vi "Make Counter Signal.vi"(11 "Node Ptr":T1=18446744073709551615 format="%.0x") -> ()   [LabVIEW 2025, in "Protection and Counter Addon System Explorer.lvlib"]
uses:
  Protection and Counter Addon System Explorer.lvlib
  Addon Shared/SubVIs/GUID Lookup.vi
  Addon Shared/Protection and Counter Addon Shared.lvlib
  SubModules/Frame-Protection-Support/Source/System Explorer/Protection and Counter Support System Explorer.lvlib
  SubModules/Frame-Protection-Support/Source/System Explorer/Types/Switch GUID Settings.ctl
  <vilib>/NI VeriStand/Custom Device API/Custom Device Item Ref.ctl
  <vilib>/NI VeriStand/Custom Device API/Custom Device API.lvlib
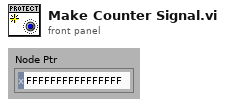
[diagram p1: front panel]
types:
  T1 = typedef "Custom Device API.lvlib/Custom Device Item Ref.ctl" = u64
  T2 = typedef "Switch GUID Settings.ctl" = cluster{"Incoming Page":string, "Protection Value":string, "Protected Signal":string, "Signal Page":string, "Invalid Count Channel":string, "Counter Value Channel":string}
  T3 = typedef "Protection and Counter Addon Shared.lvlib/XNET Settings.ctl" = cluster{"Database":refnum<k21>, "Cluster":refnum<k21>, "Port":string, "Baud rate [Bd]":u64, "Termination":u32, "CAN I/O Mode":u32, "FD Baud rate [Bd]":u64, "Priority":i32, "Use Legacy":bool, "FD ISO Mode":u32, "Default Max Counter Value":dbl, "Default Protect Type":T4, "Include All Channels":bool}
  T4 = typedef "Protection and Counter Support Shared.lvlib/Protection Type.ctl" = enum16{"Arb ID + Bytes Checksum with Inversion", "Arb ID + Bytes CRC with Inversion", "Reversed Raw Signal Checksum with Inversion", "Concatenated Two's Compliment"}
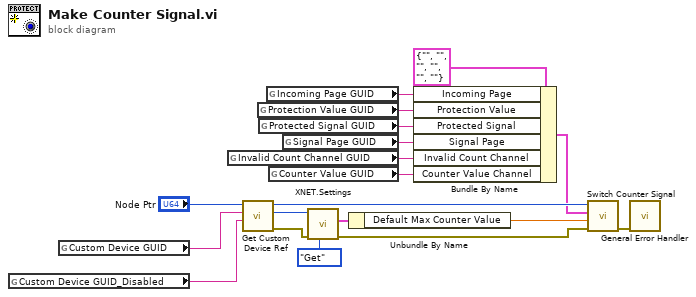
[diagram p0: block diagram]
diagram:
  n1 = global read "GUID Lookup.vi" "Custom Device GUID_Disabled"() -> (w16:string)
  n2 = global read "GUID Lookup.vi" "Custom Device GUID"() -> (w17:string)
  n3 = global read "GUID Lookup.vi" "Invalid Count Channel GUID"() -> (w5:string)
  n4 = call "Get Custom Device Ref.vi"("Custom Device GUID_Disabled"=w16, "Custom Device GUID"=w17, "Section Ptr"="Node Ptr") -> ("error out"=w14:errorcluster, "Custom Device Ref"=w12:T1, "Section Ref out"=w11:T1)  [unwired: 6 in]
  n5 = global read "GUID Lookup.vi" "Protection Value GUID"() -> (w3:string)
  n6 = global read "GUID Lookup.vi" "Protected Signal GUID"() -> (w7:string)
  n7 = global read "GUID Lookup.vi" "Incoming Page GUID"() -> (w8:string)
  n8 = global read "GUID Lookup.vi" "Counter Value GUID"() -> (w4:string)
  n9 = global read "GUID Lookup.vi" "Signal Page GUID"() -> (w6:string)
  n10 = call "XNET.Settings.vi"("Action"=enum8{"Get", "Set"}."Get", "error in (no error)"=w14, "Parent Ref in"=w12) -> ("error out"=w10:errorcluster, "XNET Settings"=w13:T3)  [unwired: 6 in, 1 out]
  n11 = Unbundle By Name(w13) -> ("Default Max Counter Value"=w1:dbl)
  n12 = Bundle By Name(cluster=T2 {"Incoming Page"="", "Protection Value"="", "Protected Signal"="", "Signal Page"="", "Invalid Count Channel"="", "Counter Value Channel"=""} ("GUIDs"), "Incoming Page"=w8, "Protection Value"=w3, "Protected Signal"=w7, "Signal Page"=w6, "Invalid Count Channel"=w5, "Counter Value Channel"=w4) -> (w2:T2)
  n13 = call "Switch Counter Signal.vi"("error in (no error)"=w10, "Default Max Count"=w1, "GUIDs"=w2, "Node Ptr"=w11) -> ("error out"=w19:errorcluster)  [unwired: 7 in]
  n14 = call <vilib>:"General Error Handler.vi"("error in (no error)"=w19) -> ()  [unwired: 10 in, 5 out]
